vi "Use the Robot Image's Add-ons.vi"() -> ()   [LabVIEW 2023]
panel:
  out "Status":string
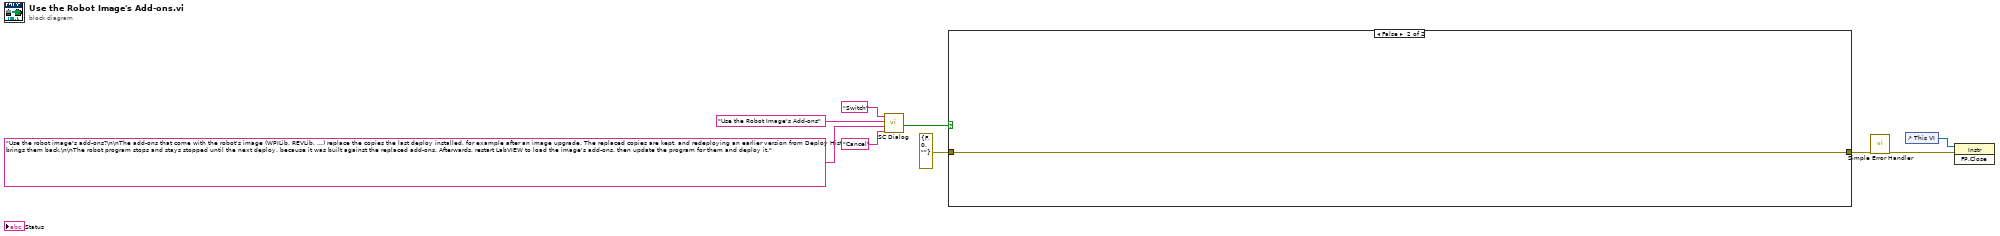
[diagram p0: block diagram]
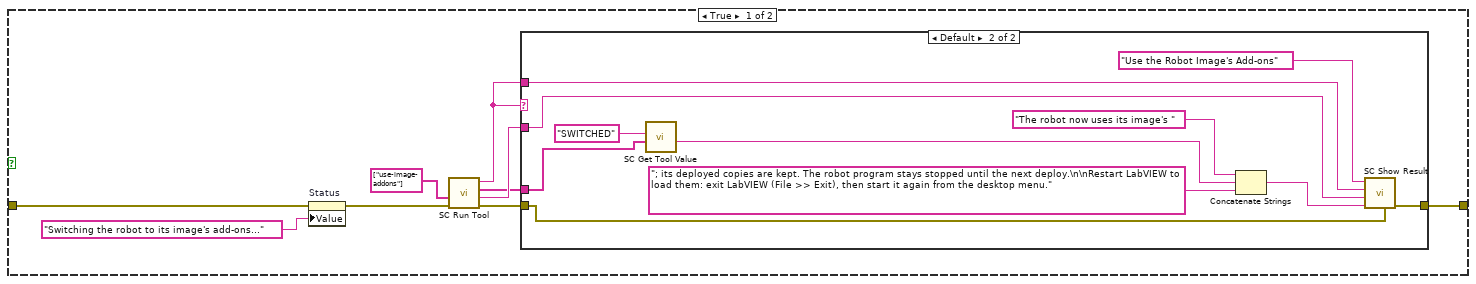
[diagram p2: hidden frame]
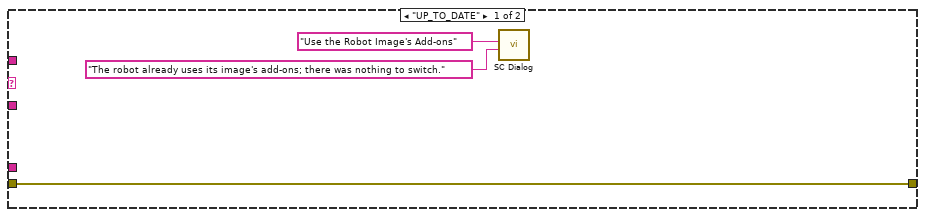
[diagram p3: hidden frame]
diagram:
  n1 = call "SC Dialog.vi"("Cancel text"="Cancel", "message"="Use the robot image's add-ons?\n\nThe add-ons that come with the robot's image (WPILib, REVLib, ...) replace the copies the last deploy installed, for example after an image upgrade. The replaced copies are kept, and redeploying an earlier version from Deploy History brings them back.\n\nThe robot program stops and stays stopped until the next deploy, because it was built against the replaced add-ons. Afterwards, restart LabVIEW to load the image's add-ons, then update the program for them and deploy it.", "window title"="Use the Robot Image's Add-ons", "OK text"="Switch") -> ("OK?"=w4:bool)  [unwired: 7 in]
  n2 = case shown="False" w4 {
    tunnel: errorcluster {"status"=FALSE, "code"=0, "source"=""} -> [w18 w33]
    tunnel: [w10 w33] -> w3
    frame True {
      n3 = property on="Status" class="Str"(error in=w18, "Value"="Switching the robot to its image's add-ons...") -> (error out=w15:errorcluster)  [unwired: 1 in, 1 out]
      n4 = call <vilib>:"SC Run Tool.vi"("error in (no error)"=w15, "arguments"=string[] ["use-image-addons"]) -> ("error out"=w14:errorcluster, "output"=w13:string, "tool lines"=w12:string[], "result"=w11:string)  [unwired: 4 in, 2 out]
      n5 = case shown="Default" w11 {
        tunnel: w14 -> [w19 w23]
        tunnel: w13 -> [_ w25]
        tunnel: w11 -> [_ w26]
        tunnel: w12 -> [_ w31]
        tunnel: [w19 w22] -> w10
        frame "UP_TO_DATE" {
          n6 = call "SC Dialog.vi"("message"="The robot already uses its image's add-ons; there was nothing to switch.", "window title"="Use the Robot Image's Add-ons") -> ()  [unwired: 9 in, 1 out]
        }
        frame Default {
          n7 = call <vilib>:"SC Get Tool Value.vi"("tool lines"=w31, "key"="SWITCHED") -> ("value"=w29:string)  [unwired: 8 in, 1 out]
          n8 = Concatenate Strings("The robot now uses its image's ", w29, "; its deployed copies are kept. The robot program stays stopped until the next deploy.\n\nRestart LabVIEW to load them: exit LabVIEW (File >> Exit), then start it again from the desktop menu.") -> (w24:string)
          n9 = call <vilib>:"SC Show Result.vi"("error in (no error)"=w23, "OK message"=w24, "output"=w25, "result"=w26, "title"="Use the Robot Image's Add-ons") -> ("error out"=w22:errorcluster)  [unwired: 6 in]
        }
      }
    }
    frame False {
    }
  }
  n10 = call <vilib>:"Simple Error Handler.vi"("error in (no error)"=w3) -> ("error out"=w1:errorcluster)  [unwired: 4 in, 4 out]
  n11 = control-ref of="This VI"() -> (w2:refnum<vi>)
  n12 = invoke class="Instr" method="FP.Close"(reference=w2, error in=w1) -> ()  [unwired: 1 in, 3 out]
